vi "Write Acyclic Tx Channel.vi"(5 "Transfer ID map":map{u32, u32}(c390), 6 "data with trigger in":T1[](array[typedef]), 7 "Acyclic Frame IDs in":u32[](array[numeric]), 8 "error in":errorcluster, 9 "labels settings for RT":T2[](array[typedef]) {"Label Timestamp Channel Data Reference" format="%.0x"; "Word Initial Raw Value" format="%032.0f"; "Label Disable/Trigger Channel Reference" format="%.0x"; "parameter driver data"."Tx parameter refs" format="%.0x"; "SDI" format="%02b"; "label" format="%.0o"}, 10 "channel number in":u8, 11 "board handle in":u8) -> (0 "error out":errorcluster, 2 "channel number out":u8, 3 "board handle out":u8)   [LabVIEW 2020, in "AIM ARINC 429 Hardware API.lvlib"]
uses:
  AIM ARINC 429 Hardware API.lvlib
  Shared/RT Label Settings.ctl
  Shared/Label.ctl
  Shared/RT Parameters.ctl
  Shared/Parameter Definition.ctl
  <vilib>/NI/NI VeriStand Encoding and Decoding/Encoding.ctl
  <vilib>/NI VeriStand/Custom Device API/Custom Device Item Ref.ctl
  Shared/Transfer Type.ctl
  <vilib>/NI VeriStand/Custom Device API/Data Reference.ctl
  Data Word with Trigger.ctl
  <instrlib>/AIM GmbH/_ARINC-429/subvi/Error Converter (ErrCode or Status).vi
  <instrlib>/AIM GmbH/_ARINC-429/subvi/Get Library Path.vi
  <instrlib>/AIM GmbH/_ARINC-429/VIs/Library/Api429Lib Error Desc Get.vi
  <instrlib>/AIM GmbH/_ARINC-429/subvi/Get Error Number Offset.vi
  <vilib>/Utility/error.llb/Error Cluster From Error Code.vi
  <instrlib>/AIM GmbH/_ARINC-429/AIM429LV.lvlib
  <vilib>/NI/NI VeriStand Encoding and Decoding/Encoding and Decoding.lvlib
  <vilib>/NI VeriStand/Custom Device API/Custom Device API.lvlib
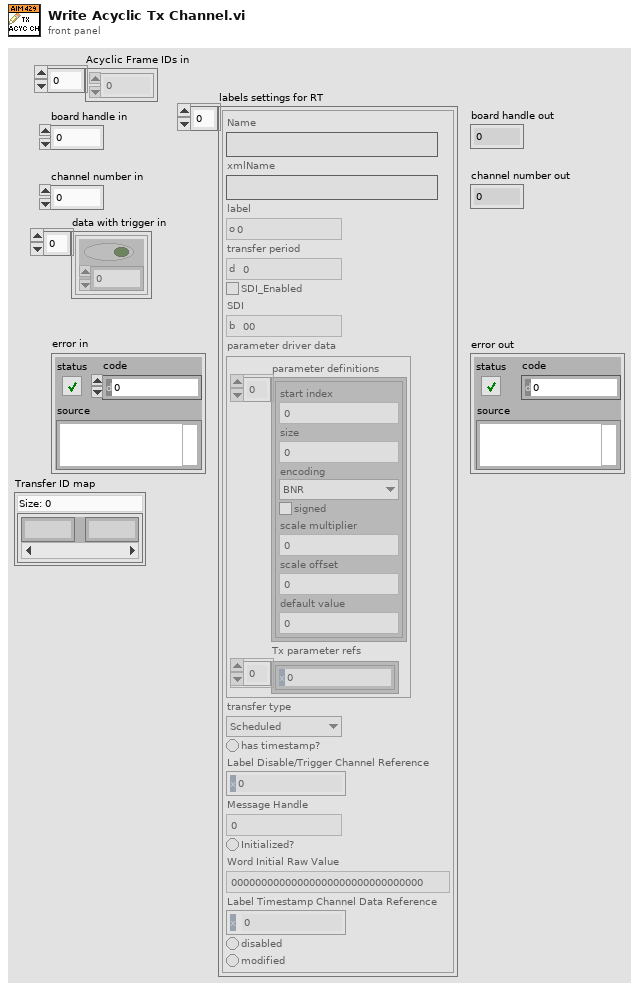
[diagram p1: front panel]
types:
  T1 = typedef "AIM ARINC 429 Hardware API.lvlib/Data Word with Trigger.ctl" = cluster{"Trigger":bool, "Data Word":u32}
  T2 = typedef "RT Label Settings.ctl" = cluster{"Name":string, "xmlName":string, "label":T3, "transfer period":u32, "SDI_Enabled":bool, "SDI":u8, "parameter driver data":T4, "transfer type":T8, "has timestamp?":bool, "Label Disable/Trigger Channel Reference":T7, "Message Handle":u64, "Initialized?":bool, "Word Initial Raw Value":u32, "Label Timestamp Channel Data Reference":T9, "disabled":bool, "modified":bool}
  T3 = typedef "Label.ctl" = u8
  T4 = typedef "RT Parameters.ctl" = cluster{"parameter definitions":T5[], "Tx parameter refs":T7[]}
  T5 = typedef "Parameter Definition.ctl" = cluster{"start index":i32, "size":i32, "encoding":T6, "signed":bool, "scale multiplier":dbl, "scale offset":dbl, "default value":dbl}
  T6 = typedef "Encoding and Decoding.lvlib/Encoding.ctl" = enum16{"BNR", "BCD", "Discrete"}
  T7 = typedef "Custom Device API.lvlib/Custom Device Item Ref.ctl" = u64
  T8 = typedef "Transfer Type.ctl" = enum16{"Scheduled", "Acyclic", "Block", "Strobe"}
  T9 = typedef "Custom Device API.lvlib/Data Reference.ctl" = i32
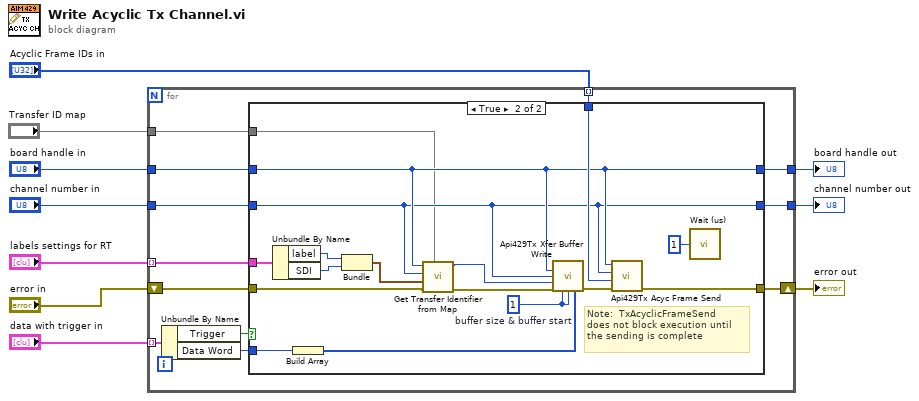
[diagram p0: block diagram]
diagram:
  n1 = for {
    tunnel: "board handle in" -> [w18]
    tunnel: "channel number in" -> [w19]
    tunnel: "labels settings for RT" -> [w22] mode=indexing
    shift-right: [w20] -> w5
    shift-left: "error in" -> [w21]
    tunnel: "data with trigger in" -> [w15] mode=indexing
    tunnel: [w17] -> w4
    tunnel: [w16] -> w3
    tunnel: "Acyclic Frame IDs in" -> [w12] mode=indexing
    tunnel: "Transfer ID map" -> [w11]
    n2 = Unbundle By Name(w15) -> ("Trigger"=w13:bool, "Data Word"=w14:u32)
    n3 = case shown="True" w13 {
      tunnel: w22 -> [_ w42]
      tunnel: w21 -> [w25 w29]
      tunnel: w14 -> [_ w41]
      tunnel: [w25 w38] -> w20
      tunnel: w19 -> [w24 w31]
      tunnel: w18 -> [w23 w32]
      tunnel: [w24 w31] -> w17
      tunnel: [w23 w32] -> w16
      tunnel: w12 -> [_ w36]
      tunnel: w11 -> [_ w26]
      frame False {
        # "if no trigger was received for this label, do not write to the hardware"
      }
      frame True {
        w39 = u16 1  # buffer size & buffer start
        # "Note:  TxAcyclicFrameSend\ndoes not block execution until\nthe sending is complete"
        n4 = Unbundle By Name(w42) -> ("label"=w34:T3, "SDI"=w33:u8)
        n5 = Build Array(w41) -> (w40:u32[])
        n6 = Bundle("label"=w34, "SDI"=w33) -> (w30:cluster{"label":T3, "SDI":u8})  [unwired: 1 in]
        n7 = call "Get Transfer Identifier from Map.vi"("Transfer ID map"=w26, "error in"=w29, "label information"=w30, "channel number in"=w31, "board number in"=w32) -> ("error out"=w28:errorcluster, "Transfer ID out"=w27:u32)  [unwired: 5 in]
        n8 = call <instrlib>:"Api429Tx Xfer Buffer Write.vi"("board_handle"=w32, "b_Chn"=w31, "ul_XferId"=w27, "error in (no error)"=w28, "w_BufStart"=w39, "w_BufSize"=w39, "pl_LData"=w40) -> ("error out"=w37:errorcluster)  [unwired: 8 in]
        n9 = call <instrlib>:"Api429Tx Acyc Frame Send.vi"("error in (no error)"=w37, "ulFrameId"=w36, "ucChannel"=w31, "board_handle"=w32) -> ("error out"=w38:errorcluster)  [unwired: 7 in]
        n10 = call "Wait (us)"("Count(uSec)"=u32 1) -> ()  [unwired: 1 out]
      }
    }
  }
  "board handle out" <- w3
  "channel number out" <- w4
  "error out" <- w5
